vi "Update_Reference.vi"(6 "New Command":bool, 8 "error in (no error)":errorcluster, 9 "StatusWord":u16, 10 "ControlWord":u16 format="%.0b", 11 "SoftmotionAxis in":refnum<class "SoftmotionAxis.lvclass">) -> (0 "error out":errorcluster, 1 "StatusWord Out":u16, 3 "SoftmotionAxis out":refnum<class "SoftmotionAxis.lvclass">)   [LabVIEW 2017, in "SoftmotionAxis.lvclass"]
uses:
  SoftmotionAxis.lvclass
  Utilities/Bit Manipulation.lvlib
  <resource>/objmgr/nimcai.rc
  <resource>/objmgr/nimotion.rc
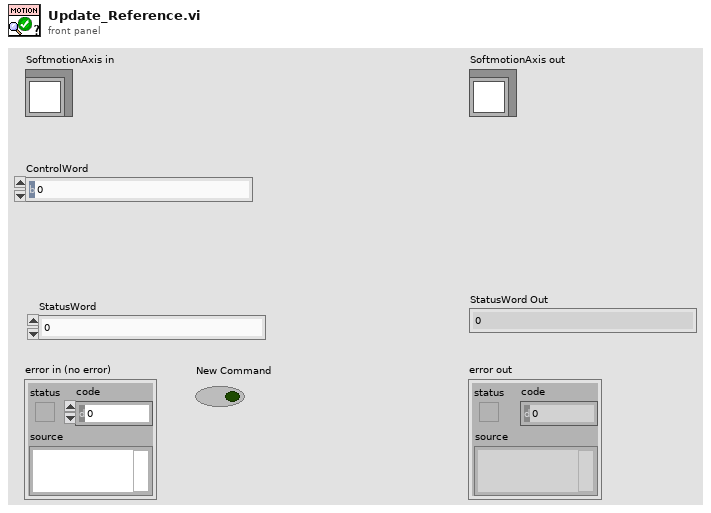
[diagram p1: front panel]
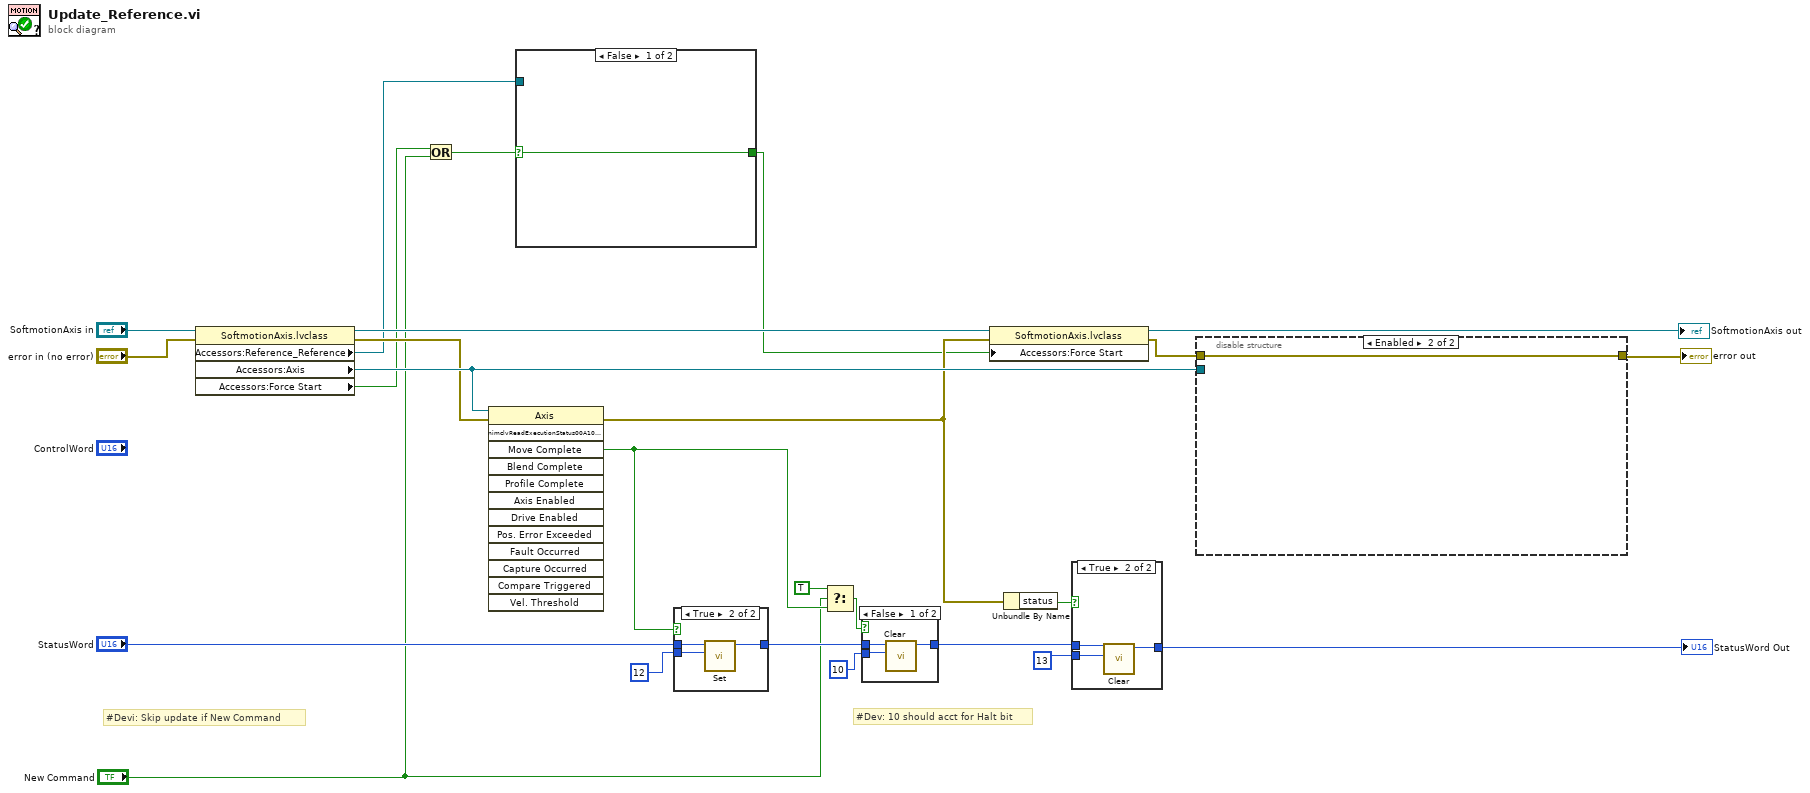
[diagram p0: block diagram]
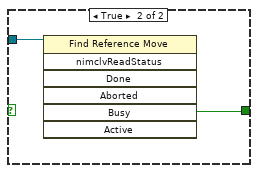
[diagram p2: hidden frame]
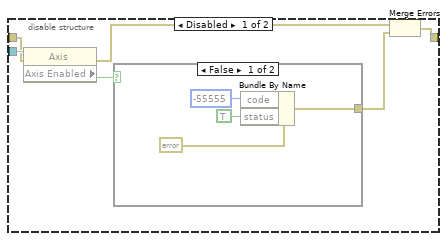
[diagram p3: hidden frame]
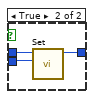
[diagram p5: hidden frame]
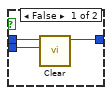
[diagram p6: hidden frame]
diagram:
  # "#Devi: Skip update if New Command"
  # "#Dev: 10 should acct for Halt bit"
  n1 = property class="SoftmotionAxis.lvclass"(reference="SoftmotionAxis in", error in="error in (no error)") -> (reference out=w22:refnum<class "SoftmotionAxis.lvclass">, error out=w10:errorcluster, "Accessors:Reference_Reference"=w5:refnum<k20>, "Accessors:Axis"=w11:refnum<k21>, "Accessors:Force Start"=w3:bool)
  n2 = Or(x=w3, y="New Command") -> (x .or. y?=w4:bool)
  n3 = invoke class="Axis" method="nimclvReadExecutionStatus00A10001"(reference=w11, error in=w10) -> (error out=w8:errorcluster, "Move Complete"=w6:bool)  [unwired: 11 in, 11 out]
  n4 = case shown="False" w4 {
    selector: w4 -> [w26 _]
    tunnel: w5 -> [_ w28]
    tunnel: [w26 w27] -> w1
    frame False {
    }
    frame True {
      n5 = invoke class="Find Reference Move" method="nimclvReadStatus"(reference=w28) -> ("Busy"=w27:bool)  [unwired: 6 in, 6 out]
    }
  }
  n6 = case shown="True" w6 {
    tunnel: u8 12 -> [w31 w34]
    tunnel: "StatusWord" -> [w30 w33]
    tunnel: [w29 w32] -> w14
    frame False {
      n7 = call "Clear.vi"("Bit to clear"=w31, "Data_In"=w30) -> ("Data_Out"=w29:u16)  [unwired: 9 in]
    }
    frame True {
      n8 = call "Set.vi"("Bit to set"=w34, "Data_In"=w33) -> ("Data_Out"=w32:u16)  [unwired: 9 in]
    }
  }
  n9 = Select(t=TRUE, s="New Command", f=w6) -> (s? t:f=w12:bool)
  n10 = case shown="False" w12 {
    tunnel: [w36 w40] -> w18
    tunnel: u8 10 -> [w35 w39]
    tunnel: w14 -> [w37 w38]
    frame False {
      n11 = call "Clear.vi"("Bit to clear"=w35, "Data_In"=w37) -> ("Data_Out"=w36:u16)  [unwired: 9 in]
    }
    frame True {
      n12 = call "Set.vi"("Bit to set"=w39, "Data_In"=w38) -> ("Data_Out"=w40:u16)  [unwired: 9 in]
    }
  }
  n13 = property class="SoftmotionAxis.lvclass"(reference=w22, error in=w8, "Accessors:Force Start"=w1) -> (reference out=→"SoftmotionAxis out":refnum<class "SoftmotionAxis.lvclass">, error out=w7:errorcluster)
  n14 = Unbundle By Name(w8) -> ("status"=w17:bool)
  n15 = case shown="True" w17 {
    tunnel: w18 -> [w41 w44]
    tunnel: [w41 w43] -> w20
    tunnel: u8 13 -> [_ w42]
    frame False {
    }
    frame True {
      n16 = call "Clear.vi"("Bit to clear"=w42, "Data_In"=w44) -> ("Data_Out"=w43:u16)  [unwired: 9 in]
    }
  }
  "StatusWord Out" <- w20
  n17 = disable-structure shown="Enabled" {
    disable-tunnel: [w47 w55] -> w24
    disable-tunnel: w11 -> [w46 _]
    disable-tunnel: w7 -> [w45 w55]
    frame Disabled {
      n18 = property class="Axis"(reference=w46, error in=w45) -> (error out=w48:errorcluster, "Axis Enabled"=w50:bool)  [unwired: 1 out]
      n19 = case shown="False" w50 {
        tunnel: [w51 _] -> w49
        frame False {
          n20 = Bundle By Name(cluster=errorcluster {"status"=FALSE, "code"=0, "source"=""} ("error in (no error)"), "code"=-55555, "status"=TRUE) -> (w51:errorcluster)
        }
        frame True {
        }
      }
      n21 = Merge Errors(w48, w49) -> (w47:errorcluster)
    }
    frame Enabled {
    }
  }
  "error out" <- w24
